vi "XPN Is Correction Ready.vi"(8 "error in (no error)":errorcluster, 10 "gainReady":i32, 11 "offsetReady":i32) -> (0 "error out":errorcluster, 1 "function return":i32, 2 "gainReady out":i32, 3 "offsetReady out":i32)   [LabVIEW 2025, in "xPanelWrapper.lvlib"]
doc: "XPN_API int XPN_IsCorrectionReady(int* offsetReady, int* gainReady);"
uses:
  xPanelWrapper.lvlib
  xPanelWrapper.dll
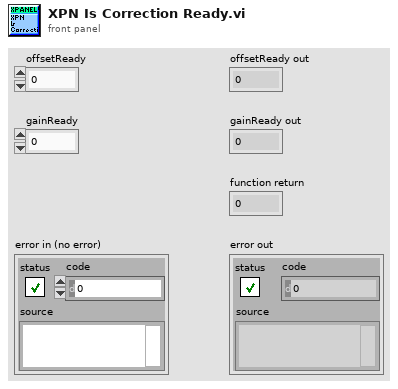
[diagram p1: front panel]
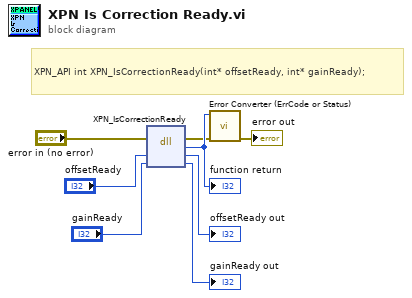
[diagram p0: block diagram]
diagram:
  # "XPN_API int XPN_IsCorrectionReady(int* offsetReady, int* gainReady);"
  n1 = dll-call lib="C:/Users/AriNutpam User/Documents/GitHub/The-Oracle/Image Acquisition/Child Classes/DTImager/xPanelWrapperLvLib/xPanelWrapper.*" fn="XPN_IsCorrectionReady"(error in="error in (no error)", "offsetReady"="offsetReady", "gainReady"="gainReady") -> (error out=w2:errorcluster, w8:i32, "offsetReady"=→"offsetReady out":i32, "gainReady"=→"gainReady out":i32)  [unwired: 2 in, 1 out]
  "function return" <- w8
  n2 = call "Error Converter (ErrCode or Status).vi"("error in (no error)"=w2, "error code"=w8) -> ("error out"=→"error out":errorcluster)  [unwired: 9 in]
